vi "Open Linear Measurement Panel.vi"(8 "error in (no error)":errorcluster caption="错误输入（无错误）", 10 "Linear Measurement Module ID":i32, 11 "Data Viewer 输入":refnum<class "Data Viewer.lvclass">) -> (0 "error out":errorcluster caption="错误输出", 3 "Data Viewer 输出":refnum<class "Data Viewer.lvclass">)   [LabVIEW 2020]
uses:
  NI/20_cRIO/Axis Controller V4/Axis Controller UI/Libraries/Data Save/Linear Measurement Panel/Linear Measurement Panel.lvlib
  Data Viewer.lvclass
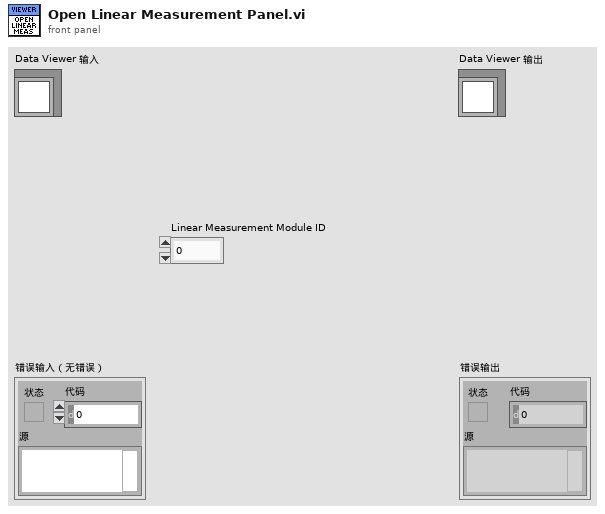
[diagram p1: front panel]
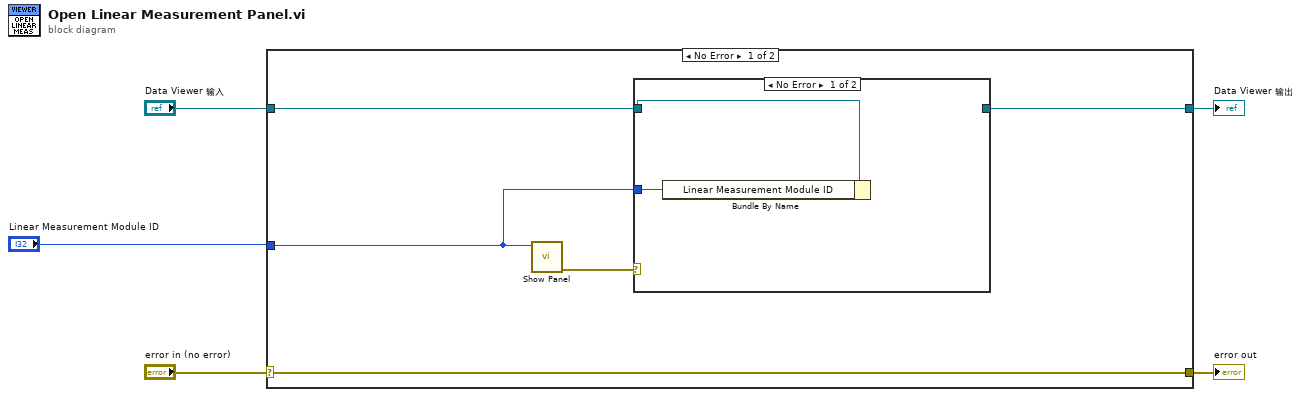
[diagram p0: block diagram]
diagram:
  n1 = case shown="No Error" "error in (no error)" {
    selector: "error in (no error)" -> [w10 w15]
    tunnel: [w10 w15] -> w4
    tunnel: [w8 w14] -> w2
    tunnel: "Data Viewer 输入" -> [w9 w14]
    tunnel: "Linear Measurement Module ID" -> [w7 _]
    frame No Error {
      n2 = call "Show Panel.vi"("Module ID"=w7) -> ("error out"=w6:errorcluster)  [unwired: 10 in]
      n3 = case shown="No Error" w6 {
        tunnel: w9 -> [w11 w13]
        tunnel: [_ w13] -> w8
        tunnel: w7 -> [w12 _]
        frame No Error {
          n4 = Bundle By Name(cluster=w11, "Linear Measurement Module ID"=w12) -> ()  [unwired: 1 out]
        }
        frame Error {
        }
      }
    }
    frame Error {
    }
  }
  "error out" <- w4
  "Data Viewer 输出" <- w2
